vi "D_Reboot.vi"(8 "error in (no error)":errorcluster, 11 "bID":u8) -> (0 "error out":errorcluster, 3 "bID":u8)   [LabVIEW 2017]
uses:
  LabVIEW2018/hpkSLMdaLV.dll
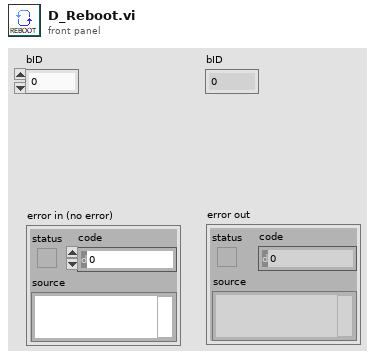
[diagram p1: front panel]
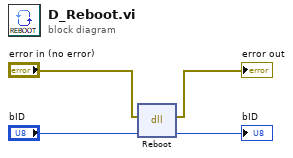
[diagram p0: block diagram]
diagram:
  n1 = dll-call lib="C:/Users/hs5921/Desktop/LabVIEW2018/hpkSLMdaLV.dll" fn="Reboot"(error in="error in (no error)", "bID"="bID") -> (error out=→"error out":errorcluster, "bID"=→"bID":u8)  [unwired: 3 in, 1 out]
